vi "plcm3UnitInfo.vi"(7 "Mode":u16(ring) items=["Dialog On Error", "no dialog - CloseUnit and Stop", "no dialog - Continue", "no dialog - Stop"], 8 "error in (no error)":errorcluster, 11 "handle in":i16=16384) -> (0 "error out":errorcluster, 2 "Unit Info":T1, 3 "handle out":i16=16384)   [LabVIEW 2010]
doc: "Returns Driver and Unit Information"
uses:
  plcm3.dll
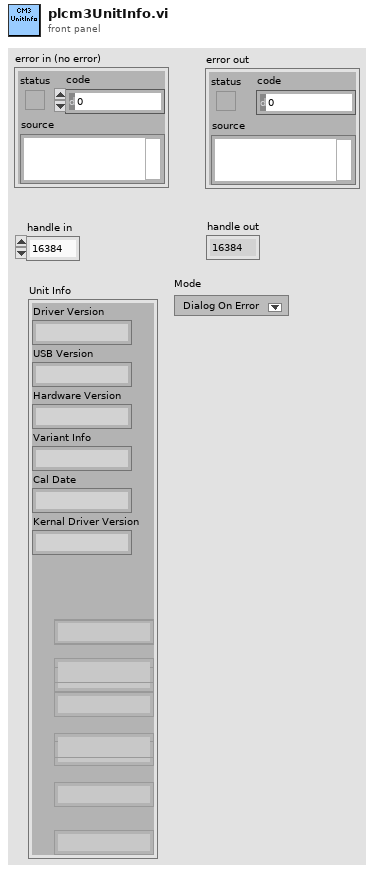
[diagram p1: front panel]
types:
  T1 = cluster{"Driver Version":string, "USB Version":string, "Hardware Version":string, "Variant Info":string, "Cal Date":string, "Kernal Driver Version":string, "NA":string, "NA 2":string, "NA":string, "NA 3":string, "NA 4":string, "NA 5":string, "NA 6":string, "NA 7":string, "NA 8":string}
  T2 = cluster{"status":bool, "code":u32, "source":string}
  T3 = cluster{"[0]":string, "[1]":string, "[2]":string, "[3]":string, "[4]":string, "[5]":string, "[6]":string, "[7]":string, "[8]":string, "[9]":string, "[10]":string, "[11]":string, "[12]":string, "[13]":string, "[14]":string}
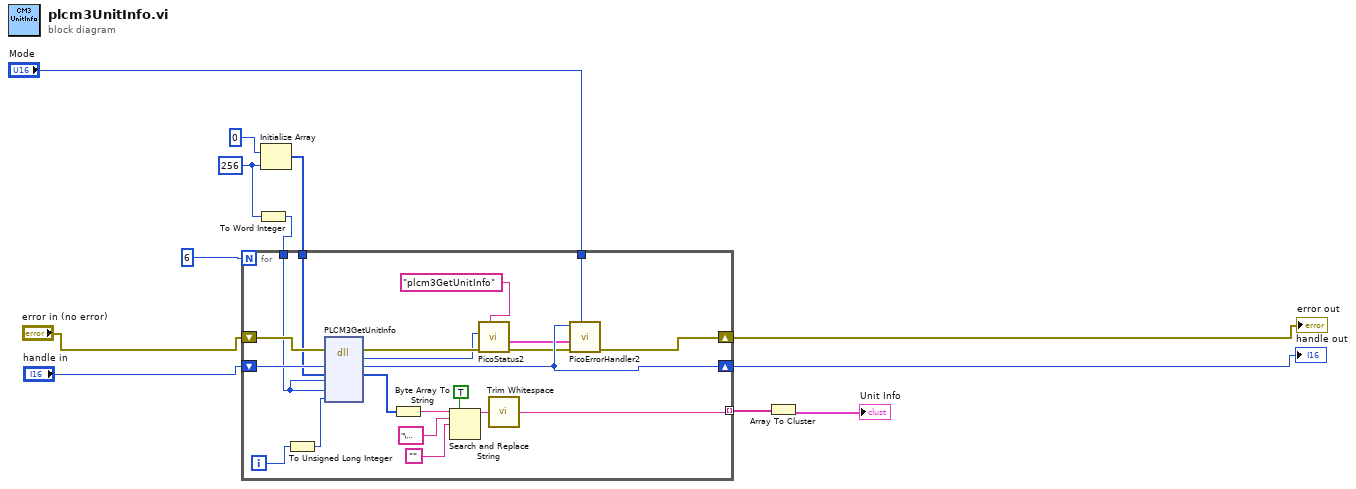
[diagram p0: block diagram]
diagram:
  w6 = 256 ("dimension size")
  n1 = To Word Integer(number=w6) -> (16bit integer=w5:i16)
  n2 = Initialize Array(u8 0 ("element"), w6) -> (w12:u8[])
  n3 = for {
    N: 6 -> [_]
    tunnel: [w20] -> w9 mode=indexing
    tunnel: w12 -> [w27]
    shift-right: [w21] -> w3
    shift-left: "handle in" -> [w29]
    shift-right: [w22] -> w4
    shift-left: "error in (no error)" -> [w28]
    tunnel: w5 -> [w19]
    tunnel: "Mode" -> [w13]
    i -> [w23]
    n4 = To Unsigned Long Integer(number=w23) -> (unsigned 32bit integer=w24:u32)
    n5 = dll-call lib="plcm3.dll" fn="PLCM3GetUnitInfo"(error in=w28, "handle"=w29, "String"=w27, "StringLength"=w19, "requiredSize"=w19, "info"=w24) -> (error out=w18:errorcluster, "PICO_STATUS"=w14:u32, "handle"=w21:i16, "String"=w26:u8[])  [unwired: 5 in, 1 out]
    n6 = Byte Array To String(unsigned byte array=w26) -> (string=w25:string)
    n7 = Search and Replace String(replace all?=TRUE ("replace all? (F)"), input string=w25, search string="\u0000", replace string="") -> (result string=w30:string)  [unwired: 4 in, 3 out]
    n8 = call "PicoStatus2.vi"("PICO source"="plcm3GetUnitInfo" ("source"), "Error in"=w18, "PICO STATUS"=w14) -> ("error out"=w16:errorcluster, "PICO_STATUS out"=w15:T2)  [unwired: 5 in]
    n9 = call <vilib>:"Trim Whitespace.vi"("string"=w30) -> ("trimmed string"=w20:string)  [unwired: 1 in]
    n10 = call "PicoErrorHandler2.vi"("Mode"=w13, "error in (no error)"=w16, "PICO_STATUS in"=w15, "handle In"=w21) -> ("error out"=w22:errorcluster)  [unwired: 7 in]
  }
  "error out" <- w4
  "handle out" <- w3
  n11 = Array To Cluster(array=w9) -> (cluster=→"Unit Info":T3)
